vi "Compile Engine Init.vi"(8 "error in (no error)":errorcluster, 11 "Device Item Ref in":T2 format="%.0x") -> (0 "error out":errorcluster, 2 "System":T1, 3 "Device Item Ref out":T2 format="%.0x")   [LabVIEW 2015, in "Engine Simulation Toolkit System Explorer.lvlib"]
uses:
  Engine Simulation Toolkit System Explorer.lvlib
  <vilib>/NI Veristand/Custom Device API/Custom Device Item Ref.ctl
  Shared/Engine Init Data.ctl
  <vilib>/NI Veristand/Custom Device API/Custom Device Channel Type.ctl
  Shared/Properties.vi
  <vilib>/NI Veristand/Custom Device API/Get Item Property (I32).vi
  <vilib>/NI Veristand/Custom Device API/Get Item Property (String).vi
  <vilib>/NI Veristand/Custom Device API/Get Item Property (Boolean).vi
  <vilib>/NI Veristand/Custom Device API/Get Item Property (Dependent File).vi
  Shared/Engine Simulation Toolkit Shared.lvlib
  <vilib>/NI Veristand/Custom Device API/Custom Device API.lvlib
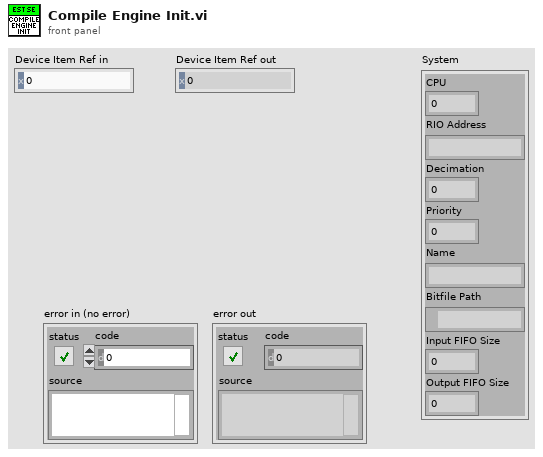
[diagram p1: front panel]
types:
  T1 = typedef "Engine Simulation Toolkit Shared.lvlib/Engine Init Data.ctl" = cluster{"CPU":i32, "RIO Address":string, "Decimation":i64, "Priority":i32, "Name":string, "Bitfile Path":path, "Input FIFO Size":i32, "Output FIFO Size":i32}
  T2 = typedef "Custom Device API.lvlib/Custom Device Item Ref.ctl" = u64
  T3 = typedef "Custom Device API.lvlib/Custom Device Channel Type.ctl" = enum16{"Input", "Output"}
  T4 = typedef "Custom Device API.lvlib/Custom Device Timed Loop Priority.ctl" = enum32{"Low", "Medium", "High"}
  T5 = typedef "Custom Device API.lvlib/Custom Device Item Info.ctl" = cluster{"Name":string, "Is Channel":bool, "GUID":string, "Is Waveform":bool}
  T6 = typedef "Custom Device API.lvlib/Dependent File Optional Info.ctl" = cluster{"Version":string, "RTDestination":path, "ForceDownload":bool, "SupportedTarget":string, "MD5":string}
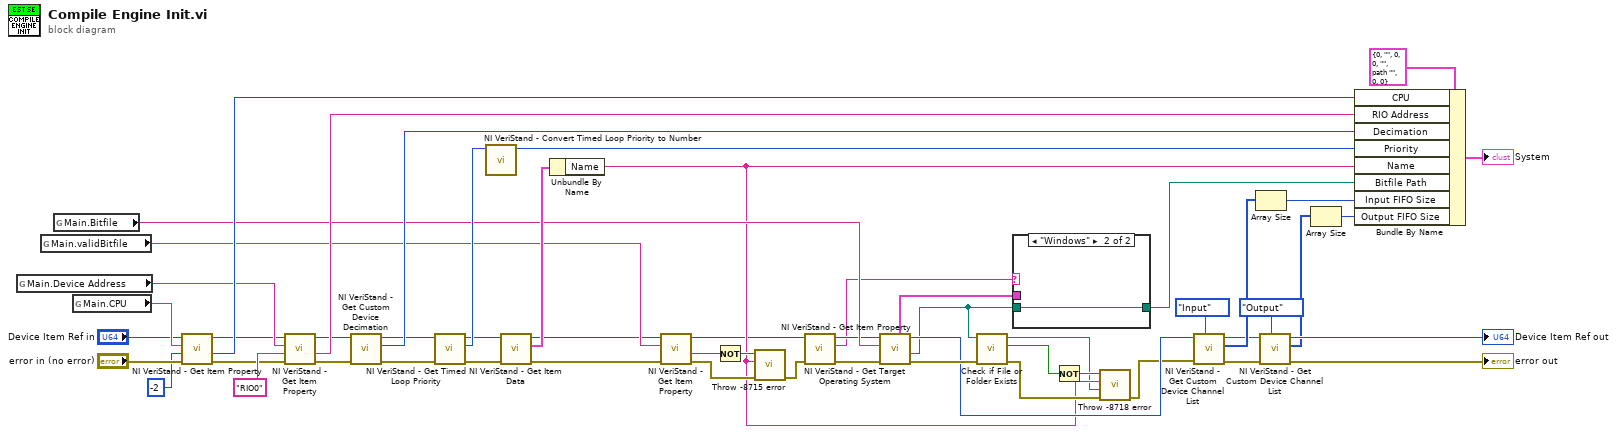
[diagram p0: block diagram]
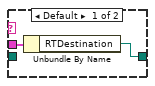
[diagram p2: hidden frame]
diagram:
  n1 = global read "Properties.vi" "Main.Device Address"() -> (w49:string)
  n2 = global read "Properties.vi" "Main.validBitfile"() -> (w33:string)
  n3 = global read "Properties.vi" "Main.Bitfile"() -> (w30:string)
  n4 = global read "Properties.vi" "Main.CPU"() -> (w53:string)
  n5 = call-poly <vilib>:"NI VeriStand - Get Item Property.vi"("error in (no error)"="error in (no error)", "Default Value"=-2, "Property Name"=w53, "Item Ref in"="Device Item Ref in") -> ("error out"=w47:errorcluster, "Value"=w51:i32, "Item Ref out"=w48:T2)  [unwired: 4 in, 1 out]
  n6 = call-poly <vilib>:"NI VeriStand - Get Item Property.vi"("error in (no error)"=w47, "Default Value"="RIO0", "Property Name"=w49, "Item Ref in"=w48) -> ("error out"=w46:errorcluster, "Value"=w45:string, "Item Ref out"=w43:T2)  [unwired: 4 in, 1 out]
  n7 = call <vilib>:"NI VeriStand - Get Custom Device Decimation.vi"("error in (no error)"=w46, "Device Ref in"=w43) -> ("error out"=w44:errorcluster, "Decimation"=w42:i32, "Device Ref out"=w40:T2)  [unwired: 7 in]
  n8 = call <vilib>:"NI VeriStand - Get Timed Loop Priority.vi"("error in (no error)"=w44, "Device Ref in"=w40) -> ("error out"=w41:errorcluster, "Priority"=w39:T4, "Device Ref out"=w37:T2)  [unwired: 7 in]
  n9 = call <vilib>:"NI VeriStand - Convert Timed Loop Priority to Number.vi"("Priority"=w39) -> ("Numeric Priority"=w38:i32)  [unwired: 10 in]
  n10 = call <vilib>:"NI VeriStand - Get Item Data.vi"("error in (no error)"=w41, "Item Ref in"=w37) -> ("error out"=w27:errorcluster, "Item Info"=w36:T5, "Item Ref out"=w26:T2)  [unwired: 6 in, 1 out]
  n11 = Unbundle By Name(w36) -> ("Name"=w8:string)
  n12 = call-poly <vilib>:"NI VeriStand - Get Item Property.vi"("error in (no error)"=w27, "Property Name"=w33, "Item Ref in"=w26) -> ("error out"=w31:errorcluster, "Value"=w32:bool, "Item Ref out"=w3:T2)  [unwired: 5 in, 1 out]
  n13 = Not(x=w32) -> (.not. x?=w15:bool)
  n14 = call "Throw -8715 error.vi"("error in (no error)"=w31, "Custom device name"=w8, "Error"=w15) -> ("error out"=w5:errorcluster)  [unwired: 8 in]
  n15 = call "NI VeriStand - Get Target Operating System.vi"("error in (no error)"=w5, "Item Ref in"=w3) -> ("error out"=w4:errorcluster, "Operating System Name"=w1:string, "Item Ref out"=w2:T2)  [unwired: 7 in]
  n16 = call-poly <vilib>:"NI VeriStand - Get Item Property.vi"("error in (no error)"=w4, "Property Name"=w30, "Item Ref in"=w2) -> ("error out"=w35:errorcluster, "Path"=w13:path, "Item Ref out"=w14:T2, "OptionalInfo"=w29:T6)  [unwired: 4 in, 1 out]
  n17 = call <vilib>:"Check if File or Folder Exists.vi"("error in (no error)"=w35, "path"=w13) -> ("error out"=w12:errorcluster, "file or folder exists?"=w10:bool, "dup path"=w7:path)  [unwired: 7 in]
  n18 = case shown="\"Windows\"" w1 {
    tunnel: w29 -> [w57 _]
    tunnel: w13 -> [_ w58]
    tunnel: [w56 w58] -> w6
    frame Default {
      n19 = Unbundle By Name(w57) -> ("RTDestination"=w56:path)
    }
    frame "Windows" {
    }
  }
  n20 = Not(x=w10) -> (.not. x?=w9:bool)
  n21 = call "Throw -8718 error.vi"("error in (no error)"=w12, "path"=w7, "Custom device name"=w8, "Error"=w9) -> ("error out"=w11:errorcluster)  [unwired: 7 in]
  n22 = call <vilib>:"NI VeriStand - Get Custom Device Channel List.vi"("Channel Type"=Custom_Device_Channel_Type."Input", "error in (no error)"=w11, "Device Ref in"=w14) -> ("error out"=w25:errorcluster, "Specified Channel Ref List"=w23:T2[], "Device Ref out"=w20:T2)  [unwired: 6 in]
  n23 = Array Size(array=w23) -> (size(s)=w22:i32)
  n24 = call <vilib>:"NI VeriStand - Get Custom Device Channel List.vi"("Channel Type"=Custom_Device_Channel_Type."Output", "error in (no error)"=w25, "Device Ref in"=w20) -> ("error out"=→"error out":errorcluster, "Specified Channel Ref List"=w17:T2[], "Device Ref out"=→"Device Item Ref out":T2)  [unwired: 6 in]
  n25 = Array Size(array=w17) -> (size(s)=w16:i32)
  n26 = Bundle By Name(cluster=T1 {"CPU"=0, "RIO Address"="", "Decimation"=0, "Priority"=0, "Name"="", "Bitfile Path"=path "", "Input FIFO Size"=0, "Output FIFO Size"=0} ("System"), "CPU"=w51, "RIO Address"=w45, "Decimation"=w42, "Priority"=w38, "Name"=w8, "Bitfile Path"=w6, "Input FIFO Size"=w22, "Output FIFO Size"=w16) -> (→"System":T1)
